vi "FlatToRichcif_can_writer_nixnet_XnetDevice.vi"(5 "OutputClusterType":T1, 11 "InputCluster":T2) -> (3 "OutputCluster":T1)   [LabVIEW 2021, in "CanWriterNixnet_server.lvlib"]
uses:
  CanWriterNixnet_server.lvlib
  cif_can_writer_nixnet_XnetDevice_Flat.ctl
  cif_can_writer_nixnet_XnetDevice.ctl
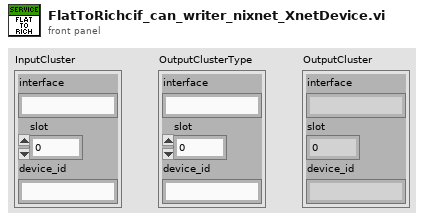
[diagram p1: front panel]
types:
  T1 = typedef "CanWriterNixnet_server.lvlib/cif_can_writer_nixnet_XnetDevice.ctl" = cluster{"interface":string, "slot":u32, "device_id":string}
  T2 = typedef "CanWriterNixnet_server.lvlib/cif_can_writer_nixnet_XnetDevice_Flat.ctl" = cluster{"interface":string, "slot":u32, "device_id":string}
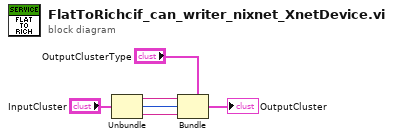
[diagram p0: block diagram]
diagram:
  n1 = Unbundle "Unbundle"("InputCluster") -> ("interface"=w3:string, "slot"=w2:u32, "device_id"=w1:string)
  n2 = Bundle "Bundle"(cluster="OutputClusterType", "interface"=w3, "slot"=w2, "device_id"=w1) -> (→"OutputCluster":T1)
